vi "FuncVI-scandbl.vi"(5 "InstanceRef":T2, 9 "arg list":T1[](array[typedef]) {"num" format="%.2f"}) -> (0 "error out":bool, 3 "result":T1 {"num" format="%.2f"})   [LabVIEW 2021]
doc: "::: CalcExpress Toolkit :::\nCopyright (c) 2000-2026 Konstantin Shifershteyn. All rights reserved."
uses:
  cetypes.llb/CalcExpress Function Argument Info.ctl
  cetypes.llb/CalcExpress Instance RefNum.ctl
panel:
  in  "max arg num":i32=3
  in  "min arg num":i32=1
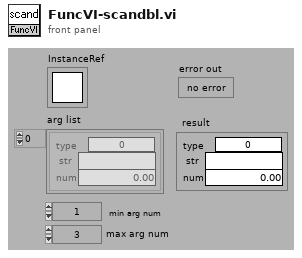
[diagram p1: front panel]
types:
  T1 = typedef "CalcExpress Function Argument Info.ctl" = cluster{"type":u32, "str":string, "num":dbl}
  T2 = typedef "CalcExpress Instance RefNum.ctl" = refnum<k1>
  T3 = cluster{"index":i32, "data type":enum32{"String", "DBL Number", "identifier", "1D Array of DBL", "2D Array of DBL", "CDB Number", "1D Array of CDB", "2D Array of CDB", "1D Array of String", "2D Array of String", "Unknown data type"}, "default num":dbl, "default str":string}[]
  T4 = enum32{"String", "DBL Number", "identifier", "1D Array of DBL", "2D Array of DBL", "CDB Number", "1D Array of CDB", "2D Array of CDB", "1D Array of String", "2D Array of String", "Unknown data type"}
  T5 = cluster{"data type":enum32{"String", "DBL Number", "identifier", "1D Array of DBL", "2D Array of DBL", "CDB Number", "1D Array of CDB", "2D Array of CDB", "1D Array of String", "2D Array of String", "Unknown data type"}, string, dbl}
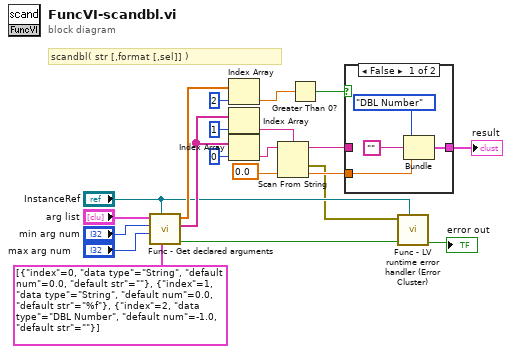
[diagram p0: block diagram]
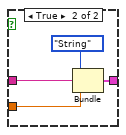
[diagram p2: hidden frame]
diagram:
  # "scandbl( str [,format [,sel]] )"
  n1 = call "Func - Get declared arguments.vi"("arg descriptors"=T3 [{"index"=0, "data type"=enum."String", "default num"=0.0, "default str"=""}, {"index"=1, "data type"=enum."String", "default num"=0.0, "default str"="%f"}, {"index"=2, "data type"=enum."DBL Number", "default num"=-1.0, "default str"=""}] ("args descriptors"), "InstanceRef"="InstanceRef", "max arg num"="max arg num", "min arg num"="min arg num", "arg list"="arg list") -> ("error out"=w4:bool, "str list"=w17:string[], "num list"=w12:dbl[])  [unwired: 3 in, 1 out]
  n2 = Index Array(array=w12, index=2) -> (element=w7:dbl)
  n3 = Index Array(array=w17, index=1) -> (element=w16:string)
  n4 = Index Array(array=w17, index=0) -> (element=w15:string)
  n5 = Scan From String(format string=w16, input string=w15, default 1=0.0) -> (remaining string=w8:string, error out=w1:errorcluster, output 1=w10:dbl)  [unwired: 2 in, 1 out]
  n6 = Greater Than 0?(x=w7) -> (x > 0?=w11:bool)
  n7 = case shown="False" w11 {
    tunnel: w10 -> [w25 w29]
    tunnel: [w22 w27] -> w9
    tunnel: w8 -> [_ w26]
    frame False {
      n8 = Bundle("data type"=T4."DBL Number", "", w25) -> (w22:T5)  [unwired: 1 in]
    }
    frame True {
      n9 = Bundle("data type"=T4."String", w26, w29) -> (w27:T5)  [unwired: 1 in]
    }
  }
  "result" <- w9
  n10 = call "Func - LV runtime error handler (Error Cluster).vi"("InstanceRef"="InstanceRef", "error in"=w4, "LabVIEW error"=w1) -> ("error out"=→"error out":bool)  [unwired: 3 in, 3 out]
